vi "Save for 2020.vi"   [LabVIEW 2023]
panel:
  # "Run me to populate the folder"
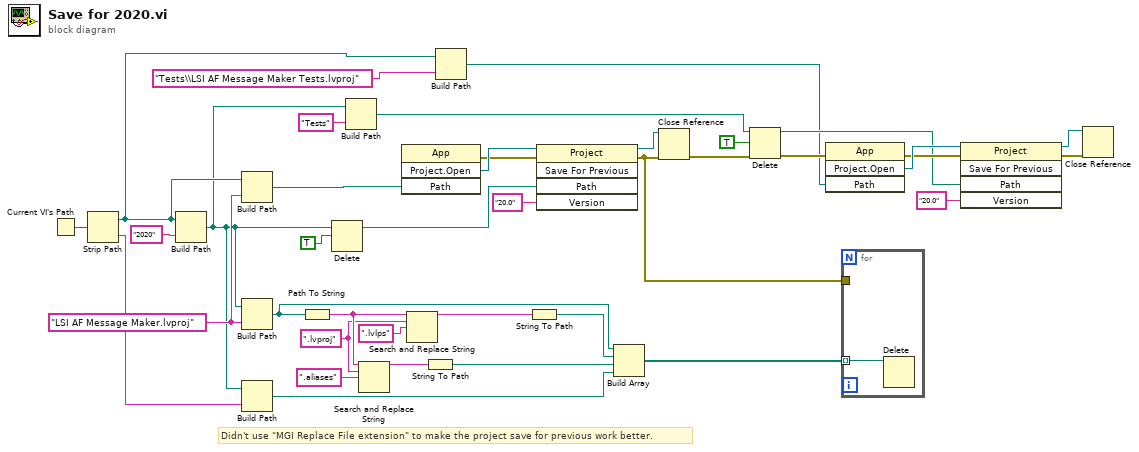
[diagram p0: block diagram]
diagram:
  w17 = ".lvproj" ("search string")
  w29 = "LSI AF Message Maker.lvproj" ("name or relative path")
  # "Didn't use \"MGI Replace File extension\" to make the project save for previous work better."
  n1 = Current VI's Path() -> (path=w38:path)
  n2 = Strip Path(path=w38) -> (stripped path=w14:path, name=w28:string)
  n3 = Build Path(base path=w14, name or relative path="2020") -> (appended path=w13:path)
  n4 = Build Path(base path=w14, name or relative path=w29) -> (appended path=w32:path)
  n5 = Build Path(base path=w13, name or relative path=w29) -> (appended path=w23:path)
  n6 = Build Path(base path=w13, name or relative path=w28) -> (appended path=w27:path)
  n7 = Path To String(path=w23) -> (string=w20:string)
  n8 = Delete(path (use dialog)=w13, entire hierarchy (F)=TRUE) -> (deleted path=w36:path)  [unwired: 3 in, 2 out]
  n9 = Build Path(base path=w13, name or relative path="Tests") -> (appended path=w9:path)
  n10 = Search and Replace String(input string=w20, search string=w17, replace string=".aliases" ("replace string (\"\")")) -> (result string=w19:string)  [unwired: 5 in, 3 out]
  n11 = invoke class="App" method="Project.Open"("Path"=w32) -> (error out=w30:errorcluster, "Project:Open"=w33:refnum<vi>)  [unwired: 3 in, 2 out]
  n12 = Search and Replace String(input string=w20, search string=w17, replace string=".lvlps" ("replace string (\"\")")) -> (result string=w22:string)  [unwired: 5 in, 3 out]
  n13 = String To Path(string=w19) -> (path=w18:path)
  n14 = Build Path(base path=w14, name or relative path="Tests\\LSI AF Message Maker Tests.lvproj") -> (appended path=w2:path)
  n15 = String To Path(string=w22) -> (path=w21:path)
  n16 = invoke class="Project" method="Save For Previous"(reference=w33, error in=w30, "Path"=w36, "Version"="20.0") -> (reference out=w31:refnum<vi>, error out=w25:errorcluster)  [unwired: 1 in, 3 out]
  n17 = Build Array(w23, w21, w18, w27) -> (w26:path[])
  n18 = Close Reference(reference=w31, error in (no error)=w25) -> (error out=w10:errorcluster)
  n19 = Delete(path (use dialog)=w9, entire hierarchy (F)=TRUE, error in=w10) -> (deleted path=w4:path, error out=w3:errorcluster)  [unwired: 2 in, 1 out]
  n20 = invoke class="App" method="Project.Open"(error in=w3, "Path"=w2) -> (error out=w6:errorcluster, "Project:Open"=w7:refnum<vi>)  [unwired: 2 in, 2 out]
  n21 = for {
    tunnel: w26 -> [w39] mode=indexing
    tunnel: w25 -> [_]
    n22 = Delete(path (use dialog)=w39) -> ()  [unwired: 4 in, 3 out]
  }
  n23 = invoke class="Project" method="Save For Previous"(reference=w7, error in=w6, "Path"=w4, "Version"="20.0") -> (reference out=w1:refnum<vi>, error out=w5:errorcluster)  [unwired: 1 in, 3 out]
  n24 = Close Reference(reference=w1, error in (no error)=w5) -> ()  [unwired: 1 out]
